vi "Update Messages MetaData.vi"(5 "enum metadata":T1[](array[typedef]), 7 "messages metadata":T2[](array[typedef]), 8 "error in (no error)":errorcluster, 11 "library in":refnum<vi>) -> (0 "error out":errorcluster, 3 "library out":refnum<vi>)   [LabVIEW 2019, in "gRPC Template Creation Utility.lvlib"]
uses:
  gRPC Template Creation Utility.lvlib
  TypeDefs/Message Metadata (Scripting).ctl
  TypeDefs/Message Element Metadata (Scripting).ctl
  TypeDefs/Message Element Type.ctl
  TypeDefs/Enum Metadata (Scripting).ctl
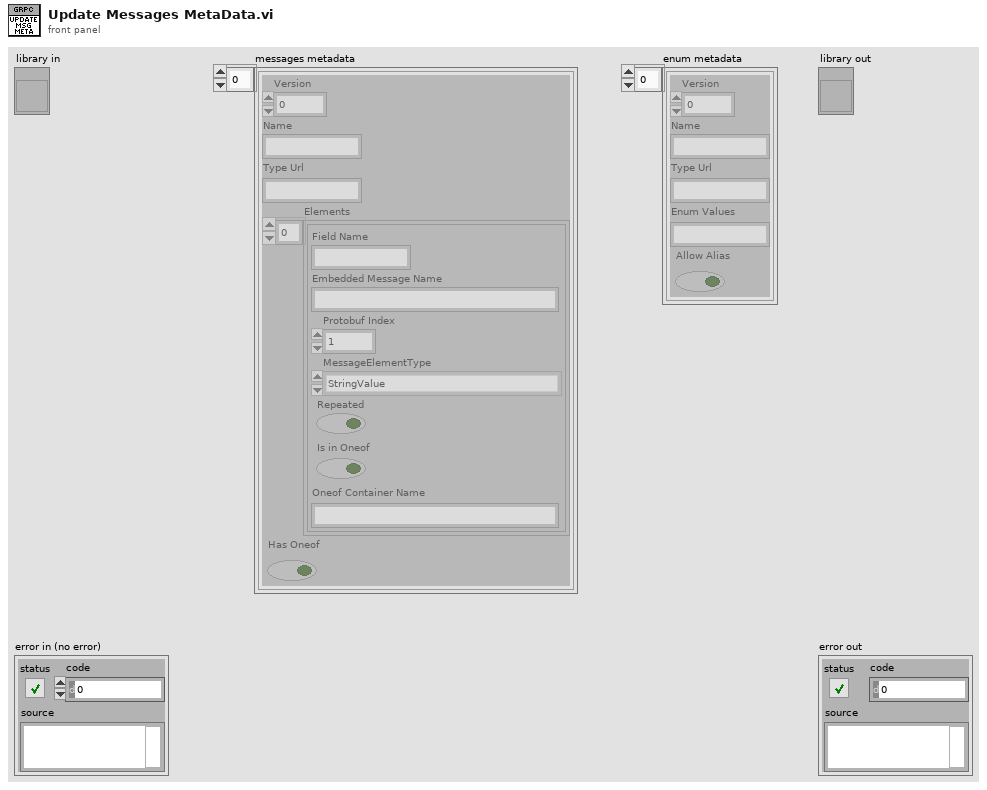
[diagram p1: front panel]
types:
  T1 = typedef "gRPC Template Creation Utility.lvlib/Enum Metadata (Scripting).ctl" = cluster{"Version":i32, "Name":string, "Type Url":string, "Enum Values":string, "Allow Alias":bool}
  T2 = typedef "gRPC Template Creation Utility.lvlib/Message Metadata (Scripting).ctl" = cluster{"Version":i32, "Name":string, "Type Url":string, "Elements":T3[], "Has Oneof":bool}
  T3 = typedef "gRPC Template Creation Utility.lvlib/Message Element Metadata (Scripting).ctl" = cluster{"Field Name":string, "Embedded Message Name":string, "Protobuf Index":i32, "MessageElementType":T4, "Repeated":bool, "Is in Oneof":bool, "Oneof Container Name":string}
  T4 = typedef "gRPC Template Creation Utility.lvlib/Message Element Type.ctl" = enum32{"Int32Value", "FloatValue", "DoubleValue", "BoolValue", "StringValue", "MessageValue", "Int64Value", "UInt32Value", "UInt64Value", "EnumValue", "Bytes", "Fixed64", "Fixed32", "SFixed64", "SFixed32", "SInt64", "SInt32"}
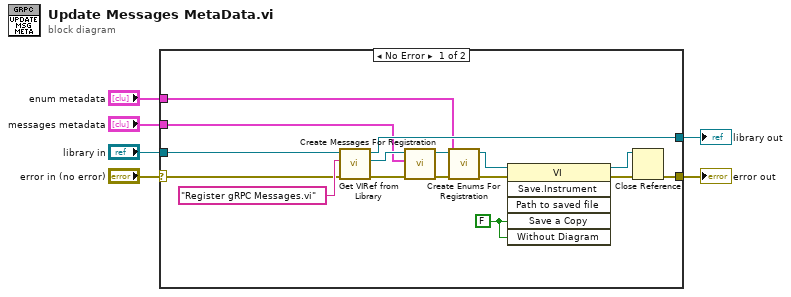
[diagram p0: block diagram]
diagram:
  n1 = case shown="No Error" "error in (no error)" {
    selector: "error in (no error)" -> [w15 w23]
    tunnel: [w22 w23] -> w6
    tunnel: [w18 w24] -> w5
    tunnel: "library in" -> [w16 w24]
    tunnel: "messages metadata" -> [w8 _]
    tunnel: "enum metadata" -> [w10 _]
    frame No Error {
      w7 = FALSE ("Save a Copy")
      n2 = call "Get VIRef from Library.vi"("error in (no error)"=w15, "item name"="Register gRPC Messages.vi" ("Item Name"), "library in"=w16) -> ("error out"=w20:errorcluster, "vi"=w19:refnum<vi>, "library out"=w18:refnum<vi>)  [unwired: 5 in, 1 out]
      n3 = call "Create Messages For Registration.vi"("error in (no error)"=w20, "Messages MetaData"=w8, "VI in"=w19) -> ("error out"=w21:errorcluster, "VI out"=w12:refnum<vi>)  [unwired: 7 in]
      n4 = call "Create Enums For Registration.vi"("error in (no error)"=w21, "Enum MetaData"=w10, "VI in"=w12) -> ("error out"=w9:errorcluster, "VI out"=w11:refnum<vi>)  [unwired: 7 in]
      n5 = invoke class="VI" method="Save.Instrument"(reference=w11, error in=w9, "Save a Copy"=w7, "Without Diagram"=w7) -> (reference out=w13:refnum<vi>, error out=w14:errorcluster)  [unwired: 2 in, 4 out]
      n6 = Close Reference(reference=w13, error in (no error)=w14) -> (error out=w22:errorcluster)
    }
    frame Error {
    }
  }
  "error out" <- w6
  "library out" <- w5
